vi "CfgManager.Collection Test Launcher.vi"() -> ()   [LabVIEW 2013]
uses:
  <vilib>/LabVIEW Open Source Project/Unicity/Delimiter/Delimiters List.ctl
  source/Manager.Text/ConfigManager.Text.lvclass
  source/Manager.Text/ConfigManager.Text.lvclass/ConfigManager.Text.ctl
  source/Collection/ConfigManagerCollection.lvclass
  <vilib>/addons/_JKI Toolkits/Caraya/classes/Assert/Assert True.vi
  source/Manager/Decompose KVPs.vi
  source/Manager/Write.vi
  source/Manager/ConfigManager.lvclass
  source/Cache/ConfigManager.Cache.lvclass
  <vilib>/LabVIEW Open Source Project/Unicity/Delimiter/Delimiter.lvclass
  <vilib>/addons/_JKI Toolkits/Caraya/classes/Test/Test.lvclass
  <vilib>/addons/_JKI Toolkits/Caraya/classes/Assert/Assert.lvclass
panel:
  out "URIs":string[](array[string])
  out "CfgManager Class Names":string[](array[string])
  out "any found? 3":bool
  out "any found?":bool
  out "any found? 2":bool
  out "modified PID settings":variant
  out "all found? 3":bool
  out "all found? 2":bool
  out "all found?":bool
  out "user-defined pump config":variant
  out "default pump config":variant
  out "default config":path
  out "merged PID settings":variant
  out "initial PID settings":variant
  out "System.Valve Keys":string[](array[string])
  out "System.Pump keys":string[](array[string])
  out "modified pump config":variant
  out "error out":errorcluster
  out "merged pump config":variant
  out "user-defined config":path
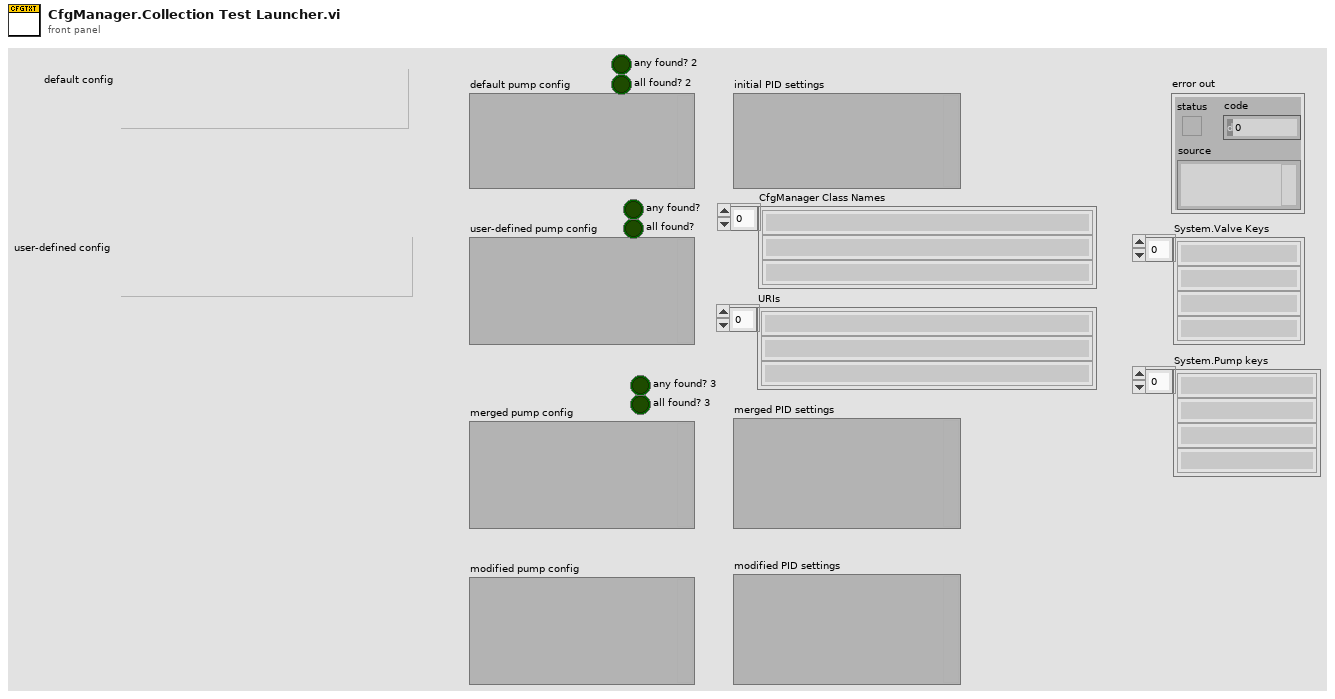
[diagram p1: front panel]
types:
  T1 = cluster{"String":string, "Numeric":dbl, "Boolean":bool}
  T2 = typedef "Delimiter.lvclass/Delimiters List.ctl" = enum16{"Default", "dot (.)", "colon (:)", "double-colon (::)", "semi-colon (;)", "underscore (_)", "double underscore (__)", "dash (-)", "double dash (--)", "backslash (\\)", "vertical bar (|)", "forward slash (/)", "chevron (>)", "double-chevron (>>)", "arrow (->)", "comma (,)", "arobas (@)", "ampersand (&)", "other"}
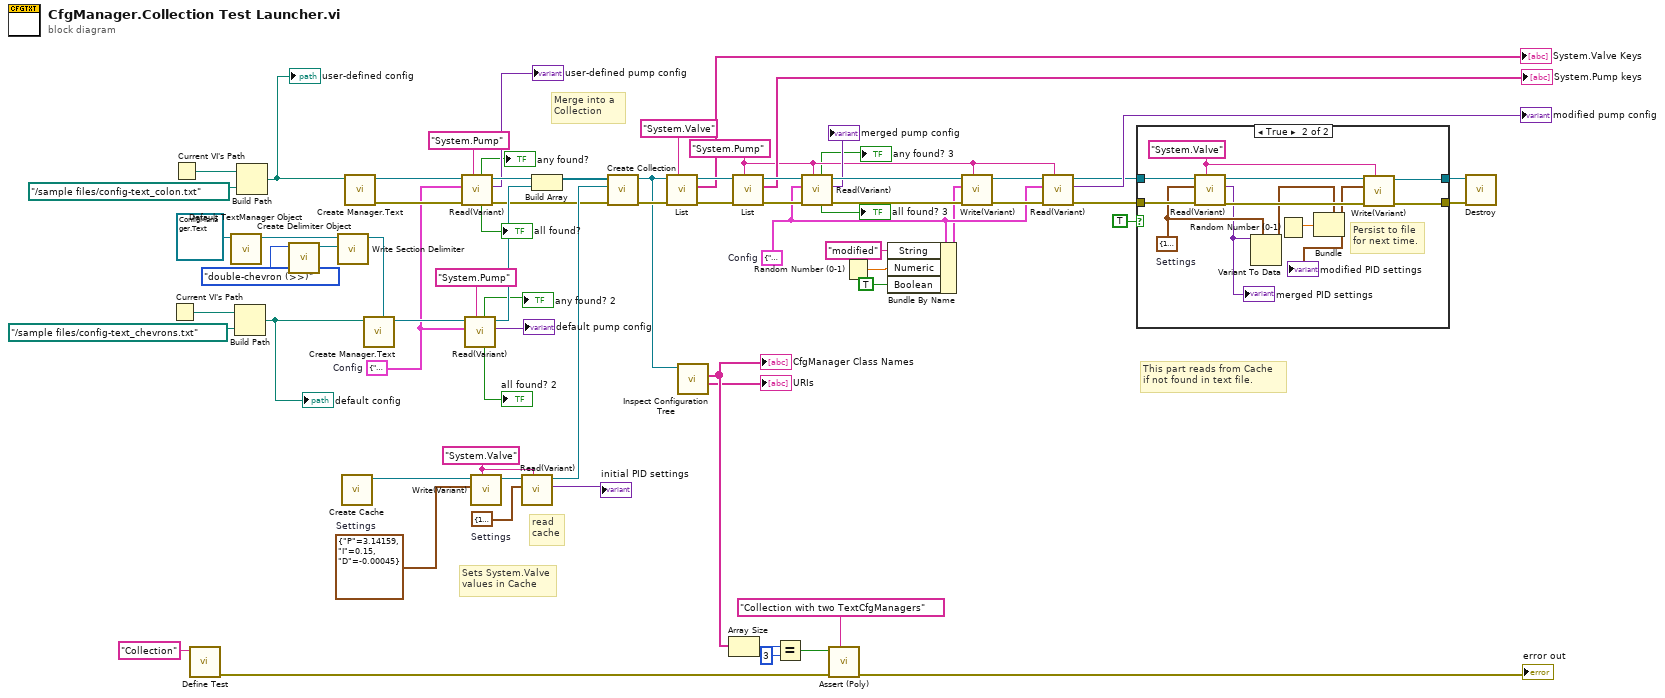
[diagram p0: block diagram]
diagram:
  w24 = T1 {"String"="", "Numeric"=0.0, "Boolean"=FALSE}  # Config
  w39 = cluster{"P":dbl, "I":dbl, "D":dbl} {"P"=1.0, "I"=0.0, "D"=0.0}  # Settings
  w54 = cluster{"P":dbl, "I":dbl, "D":dbl} {"P"=3.14159, "I"=0.15, "D"=-0.00045}  # Settings
  w40 = "System.Valve" ("Qualified Name")
  w56 = "System.Pump" ("Qualified Name")
  w55 = T1 {"String"="", "Numeric"=0.0, "Boolean"=FALSE}  # Config
  # "read\ncache"
  # "This part reads from Cache\nif not found in text file."
  # "Merge into a \nCollection"
  # "Sets System.Valve\nvalues in Cache"
  n1 = Current VI's Path() -> (path=w16:path)
  n2 = Current VI's Path() -> (path=w13:path)
  n3 = call <vilib>:"Define Test.vi"("Label (VI Title)"="Collection") -> ("error out"=w9:errorcluster)  [unwired: 10 in]
  n4 = call-dynamic "Default TextManager Object.vi"("CfgManager.Text in"=refnum<class "ConfigManager.Text.lvclass"> refnum) -> ("CfgManager.Text out"=w36:refnum<class "ConfigManager.Text.lvclass">)  [unwired: 10 in]
  n5 = Build Path(base path=w16, name or relative path=path "../sample files/config-text_chevrons.txt" ("filepath 2")) -> (appended path=w14:path)
  "default config" <- w14
  n6 = Build Path(base path=w13, name or relative path=path "../sample files/config-text_colon.txt" ("filepath 2")) -> (appended path=w11:path)
  "user-defined config" <- w11
  n7 = call <vilib>:"Create Delimiter Object.vi"("Delimiter"=Delimiters_List."double-chevron (>>)") -> ("Delimiter"=w37:refnum<class "Delimiter.lvclass">)  [unwired: 10 in]
  n8 = call "Write Section Delimiter.vi"("Section Delimiter"=w37, "ConfigManager.Text in"=w36) -> ("ConfigManager.Text out"=w35:refnum<class "ConfigManager.Text.lvclass">)  [unwired: 9 in]
  n9 = call "Create Cache.vi"() -> ("ConfigManager.Cache"=w53:refnum<class "ConfigManager.Cache.lvclass">)  [unwired: 11 in]
  n10 = call "Create Manager.Text.vi"("filepath"=w11) -> ("error out"=w29:errorcluster, "ConfigManager.Text out"=w27:refnum<class "ConfigManager.Text.lvclass">)  [unwired: 8 in, 1 out]
  n11 = call "Create Manager.Text.vi"("ConfigManager.Text"=w35, "filepath"=w14) -> ("ConfigManager.Text out"=w33:refnum<class "ConfigManager.Text.lvclass">)  [unwired: 7 in, 2 out]
  n12 = call "Read(Variant).vi"("Qualified Name"="System.Pump", "error in (no error)"=w29, "Type"=w24, "ConfigManager in"=w27) -> ("error out"=w28:errorcluster, "value"=→"user-defined pump config":variant, "ConfigManager out"=w26:refnum<class "ConfigManager.Text.lvclass">, "all found?"=→"all found?":bool, "any found?"=→"any found?":bool)  [unwired: 3 in]
  n13 = call "Read(Variant).vi"("Qualified Name"="System.Pump", "Type"=w24, "ConfigManager in"=w33) -> ("value"=→"default pump config":variant, "ConfigManager out"=w32:refnum<class "ConfigManager.Text.lvclass">, "all found?"=→"all found? 2":bool, "any found?"=→"any found? 2":bool)  [unwired: 4 in, 1 out]
  n14 = call "Write(Variant).vi"("Qualified Name"=w40, "value"=w54, "ConfigManager in"=w53) -> ("ConfigManager out"=w43:refnum<class "ConfigManager.Cache.lvclass">)  [unwired: 6 in, 2 out]
  n15 = call "Read(Variant).vi"("Qualified Name"=w40, "Type"=w39, "ConfigManager in"=w43) -> ("value"=→"initial PID settings":variant, "ConfigManager out"=w42:refnum<class "ConfigManager.Cache.lvclass">)  [unwired: 4 in, 3 out]
  n16 = Build Array(w26, w32) -> (w44:refnum<class "ConfigManager.Text.lvclass">[])
  n17 = call "Create Collection.vi"("Cache"=w42, "List"=w44) -> ("ConfigManagerCollection out"=w8:refnum<class "ConfigManagerCollection.lvclass">)  [unwired: 9 in]
  n18 = call "List.vi"("Qualified Name"="System.Valve", "error in (no error)"=w28, "ConfigManager in"=w8) -> ("error out"=w51:errorcluster, "Keys"=→"System.Valve Keys":string[], "ConfigManager out"=w52:refnum<class "ConfigManagerCollection.lvclass">)  [unwired: 6 in]
  n19 = call "Inspect Configuration Tree.vi"("ConfigManager in"=w8) -> ("URIs"=→"URIs":string[], "CfgManager Class Names"=w6:string[])  [unwired: 7 in, 2 out]
  "CfgManager Class Names" <- w6
  n20 = Array Size(array=w6) -> (size(s)=w5:i32)
  n21 = call "List.vi"("Qualified Name"=w56, "error in (no error)"=w51, "ConfigManager in"=w52) -> ("error out"=w65:errorcluster, "Keys"=→"System.Pump keys":string[], "ConfigManager out"=w64:refnum<class "ConfigManagerCollection.lvclass">)  [unwired: 6 in]
  n22 = Equal?(x=w5, y=3) -> (x = y?=w3:bool)
  n23 = call "Read(Variant).vi"("Qualified Name"=w56, "error in (no error)"=w65, "Type"=w55, "ConfigManager in"=w64) -> ("error out"=w69:errorcluster, "value"=→"merged pump config":variant, "ConfigManager out"=w70:refnum<class "ConfigManagerCollection.lvclass">, "all found?"=→"all found? 3":bool, "any found?"=→"any found? 3":bool)  [unwired: 3 in]
  n24 = call-poly <vilib>:"Assert (Poly).vi"("Label"="Collection with two TextCfgManagers", "error in (no error)"=w9, "True?"=w3) -> ("error out"=→"error out":errorcluster)  [unwired: 8 in]
  n25 = Random Number (0-1)() -> (number: 0 to 1=w46:dbl)
  n26 = Bundle By Name(cluster=w55, "String"="modified", "Numeric"=w46, "Boolean"=TRUE) -> (w45:T1)
  n27 = call "Write(Variant).vi"("Qualified Name"=w56, "error in (no error)"=w69, "value"=w45, "ConfigManager in"=w70) -> ("error out"=w67:errorcluster, "ConfigManager out"=w68:refnum<class "ConfigManagerCollection.lvclass">)  [unwired: 5 in, 1 out]
  n28 = call "Read(Variant).vi"("Qualified Name"=w56, "error in (no error)"=w67, "Type"=w55, "ConfigManager in"=w68) -> ("error out"=w59:errorcluster, "value"=→"modified pump config":variant, "ConfigManager out"=w61:refnum<class "ConfigManagerCollection.lvclass">)  [unwired: 3 in, 2 out]
  n29 = case shown="True" TRUE {
    tunnel: w61 -> [w72 w84]
    tunnel: [w72 w79] -> w60
    tunnel: w59 -> [w71 w83]
    tunnel: [w71 w78] -> w58
    frame False {
    }
    frame True {
      w77 = cluster{"P":dbl, "I":dbl, "D":dbl} {"P"=1.0, "I"=0.0, "D"=0.0}  # Settings
      w80 = "System.Valve" ("Qualified Name")
      # "Persist to file\nfor next time."
      n30 = call "Read(Variant).vi"("Qualified Name"=w80, "error in (no error)"=w83, "Type"=w77, "ConfigManager in"=w84) -> ("error out"=w81:errorcluster, "value"=w76:variant, "ConfigManager out"=w82:refnum<class "ConfigManagerCollection.lvclass">)  [unwired: 3 in, 2 out]
      "merged PID settings" <- w76
      n31 = Variant To Data(type=w77, Variant=w76) -> (data=w74:cluster{"P":dbl, "I":dbl, "D":dbl})  [unwired: 1 in, 1 out]
      n32 = Random Number (0-1)() -> (number: 0 to 1=w75:dbl)
      n33 = Bundle(cluster=w74, "I"=w75) -> (w73:cluster{"P":dbl, "I":dbl, "D":dbl})  [unwired: 2 in]
      "modified PID settings" <- w73
      n34 = call "Write(Variant).vi"("Qualified Name"=w80, "error in (no error)"=w81, "value"=w73, "ConfigManager in"=w82) -> ("error out"=w78:errorcluster, "ConfigManager out"=w79:refnum<class "ConfigManagerCollection.lvclass">)  [unwired: 5 in, 1 out]
    }
  }
  n35 = call-dynamic "Destroy.vi"("error in (no error)"=w58, "ConfigManagerCollection in"=w60) -> ()  [unwired: 8 in, 2 out]
